vi "KYFG Camera Open.vi"(8 "error in (no error)":errorcluster, 11 "camHandle":u32) -> (0 "error out":errorcluster, 3 "camHandle out":u32)   [LabVIEW 2023, in "KYFGLib_lv.lvlib"]
doc: "KYFG_API FGSTATUS KYFG_CameraOpen(CAMHANDLE camHandle, const char *xml_file_path, const char* project_file_path);"
uses:
  KYFGLib_lv.lvlib
  KYFGLib.dll
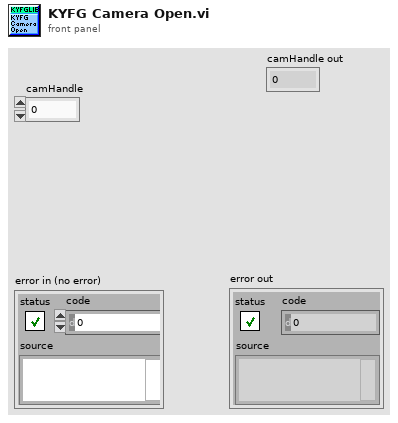
[diagram p1: front panel]
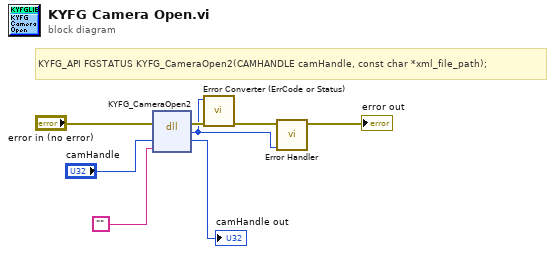
[diagram p0: block diagram]
diagram:
  # "KYFG_API FGSTATUS KYFG_CameraOpen2(CAMHANDLE camHandle, const char *xml_file_path);"
  n1 = dll-call lib="KYFGLib.dll" fn="KYFG_CameraOpen2"(error in="error in (no error)", "camHandle"="camHandle", "xml_file_path"="") -> (error out=w6:errorcluster, "return type"=w3:u32, "camHandle"=→"camHandle out":u32)  [unwired: 3 in, 1 out]
  n2 = call "Error Converter (ErrCode or Status).vi"("error in (no error)"=w6, "error code"=w3) -> ("error out"=w5:errorcluster)  [unwired: 9 in]
  n3 = call "Error Handler.vi"("Return Code"=w3, "Error In"=w5) -> ("Error Out"=→"error out":errorcluster)  [unwired: 9 in]
